vi "xnet_canopen_initialize.vi"(6 "persistence LSS path":string, 8 "error in (no error)":errorcluster, 9 "model json path":string, 10 "XNET Interface":refnum<k21>, 11 "xnet_co_handle_in":u64) -> (0 "error out":errorcluster, 3 "xnet_co_handle":u64)   [LabVIEW 2023, in "xnet_canopen.lvlib"]
uses:
  <vilib>/Utility/error.llb/Error Cluster From Error Code.vi
  xnet_canopen.lvlib
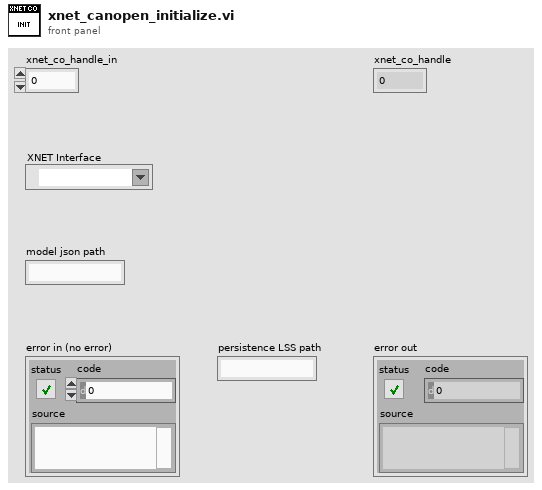
[diagram p1: front panel]
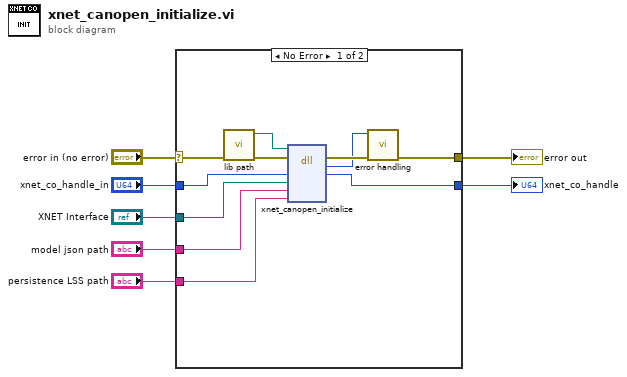
[diagram p0: block diagram]
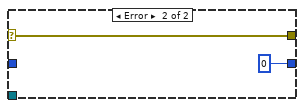
[diagram p2: hidden frame]
diagram:
  n1 = case shown="No Error" "error in (no error)" {
    selector: "error in (no error)" -> [w16 w19]
    tunnel: [w14 w19] -> w6
    tunnel: [w12 u64 0 ("phandle")] -> w5
    tunnel: "xnet_co_handle_in" -> [w11 _]
    tunnel: "XNET Interface" -> [w10 _]
    tunnel: "model json path" -> [w9 _]
    tunnel: "persistence LSS path" -> [w8 _]
    frame No Error {
      n2 = call "lib path.vi"() -> ("lib path"=w17:path)  [unwired: 11 in]
      n3 = dll-call lib="?" fn="xnet_canopen_initialize"(path in=w17, error in=w16, "handle"=w11, "xnet_port"=w10, "model_json"=w9, "persistence_lss"=w8) -> (error out=w15:errorcluster, "return type"=w13:i32, "handle"=w12:u64)  [unwired: 4 in, 1 out]
      n4 = call "error handling.vi"("error in (no error)"=w15, "return val"=w13) -> ("error out"=w14:errorcluster)  [unwired: 9 in]
    }
    frame Error {
    }
  }
  "error out" <- w6
  "xnet_co_handle" <- w5
